vi "string to system.vi"(8 "error in":errorcluster, 11 "data":string) -> (0 "error out":errorcluster, 2 "system":T1)   [LabVIEW 2014, in "PLConfigurationSerializer.lvlib"]
doc: "Converts a string of data into a full system of configuration classes. This is the parser for the TBD file."
uses:
  PLConfigurationSerializer.lvlib
  system configuration/PL_System Configuration.lvclass
  target configuration/PL_Target Configuration.lvclass
  <vilib>/NI/Module Execution Interface/Engine Configuration/engine configuration.lvclass
  <vilib>/NI/Tag Bus Module Framework/module configuration/TBM module configuration.lvclass
  engines cluster.ctl
  targets cluster.ctl
  systems cluster.ctl
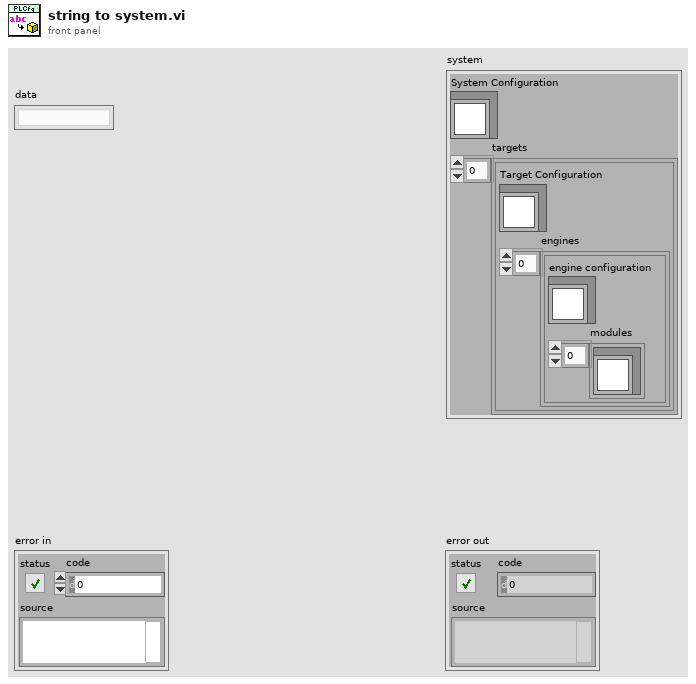
[diagram p1: front panel]
types:
  T1 = typedef "PLConfigurationSerializer.lvlib/systems cluster.ctl" = cluster{"System Configuration":refnum<class "PL_System Configuration.lvclass">, "targets":T2[]}
  T2 = typedef "PLConfigurationSerializer.lvlib/targets cluster.ctl" = cluster{"Target Configuration":refnum<class "PL_Target Configuration.lvclass">, "engines":T3[]}
  T3 = typedef "PLConfigurationSerializer.lvlib/engines cluster.ctl" = cluster{"engine configuration":refnum<class "engine configuration.lvclass">, "modules":refnum<class "TBM module configuration.lvclass">[]}
  T4 = typedef "PLConfigurationSerializer.lvlib/file format.ctl" = cluster{"version":string, "data":string}
  T5 = typedef "PLConfigurationSerializer.lvlib/1_0_0_0 format.ctl" = cluster{"system":T6, "database":T9[]}
  T6 = typedef "PLConfigurationSerializer.lvlib/system hierarchy.ctl" = cluster{"system ID":string, "targets":T7[]}
  T7 = typedef "PLConfigurationSerializer.lvlib/target hierarchy.ctl" = cluster{"target ID":string, "engines":T8[]}
  T8 = typedef "PLConfigurationSerializer.lvlib/engine hierarchy.ctl" = cluster{"engine ID":string, "modules IDs":string[]}
  T9 = typedef "PLConfigurationSerializer.lvlib/configuration database.ctl" = cluster{"ID":string, "display name":string, "class":string, "version":string, "data":string}
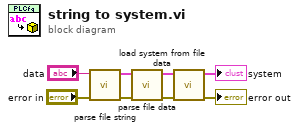
[diagram p0: block diagram]
diagram:
  n1 = call "parse file string.vi"("error in"="error in", "data string"="data") -> ("error out"=w5:errorcluster, "file format"=w6:T4)  [unwired: 8 in]
  n2 = call "parse file data.vi"("error in"=w5, "file format"=w6) -> ("error out"=w3:errorcluster, "file information"=w4:T5)  [unwired: 8 in]
  n3 = call "load system from file data.vi"("error in"=w3, "file information"=w4) -> ("error out"=→"error out":errorcluster, "system"=→"system":T1)  [unwired: 8 in]
